vi "RemoteVI Hover Parent Menu.vi"(0 "hWnd":u64, 1 "now":u32, 5 "menus":T2(array[cluster]), 7 "k":i32=1, 9 "state":T1, 11 "error in":errorcluster) -> (4 "state out":T1, 15 "error out":errorcluster)   [LabVIEW 2020, in "RemoteVI.lvlib"]
doc: "The remote pointer rests over a PARENT menu (menus[k], k > 0) while k submenus are open below it - what happens locally when the pointer moves back from a submenu. When the pointer is on the parent's highlighted item (the one that opened the submenu) nothing changes and the submenu stays open. Otherwise, once the pointer has not moved for 300 ms (so a pointer crossing the parent on its way into the submenu does not close it), the k submenus are closed with VK_LEFT (RemoteVI Close Submenus.vi) and the parent's highlight is moved under the pointer (RemoteVI Hover Navigate.vi). Before that state passes through unchanged. Win32 only, no VI Server call."
uses:
  RemoteVI.lvlib
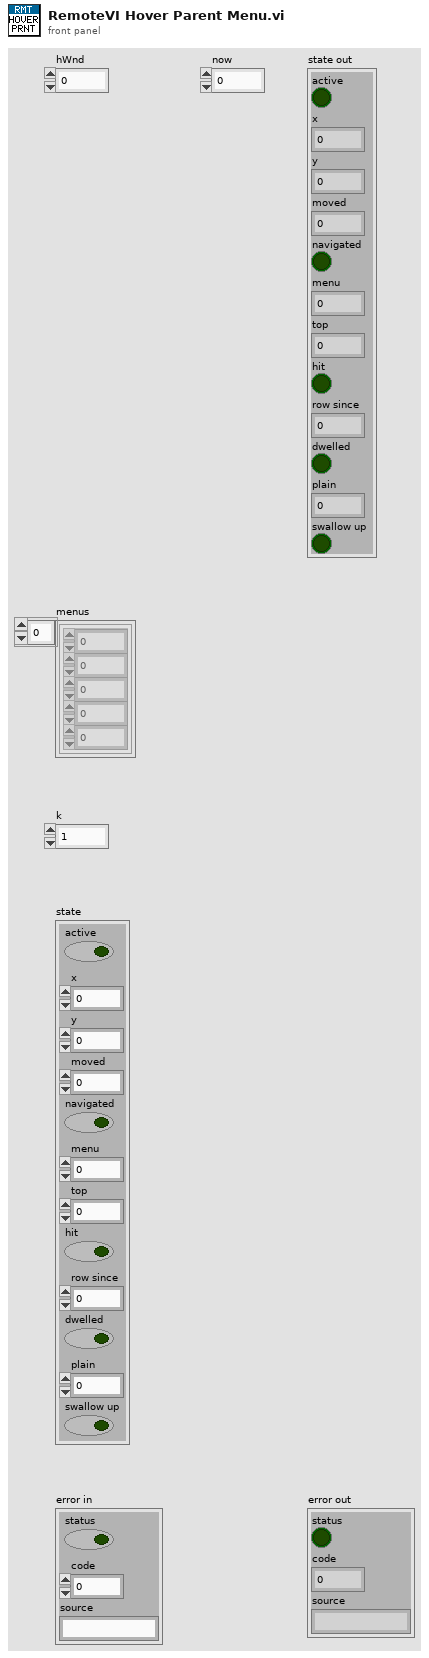
[diagram p1: front panel]
types:
  T1 = cluster{"active":bool, "x":i32, "y":i32, "moved":u32, "navigated":bool, "menu":u64, "top":i32, "hit":bool, "row since":u32, "dwelled":bool, "plain":u64, "swallow up":bool}
  T2 = cluster{"hwnd":u64, "x":i32, "y":i32, "w":i32, "h":i32}[]
  T3 = cluster{"hwnd":u64, "x":i32, "y":i32, "w":i32, "h":i32}
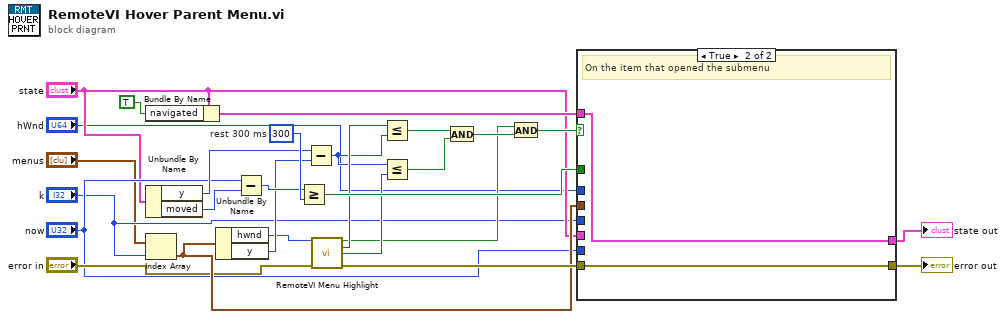
[diagram p0: block diagram]
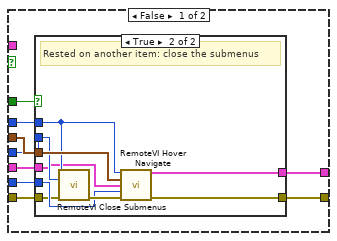
[diagram p2: hidden frame]
diagram:
  w22 = u32 300  # rest 300 ms
  n1 = Bundle By Name(cluster="state", "navigated"=TRUE) -> (w25:T1)
  n2 = Unbundle By Name("state") -> ("y"=w10:i32, "moved"=w11:u32)
  n3 = Index Array(array="menus", index="k") -> (element=w7:T3)
  n4 = Unbundle By Name(w7) -> ("hwnd"=w8:u64, "y"=w9:i32)
  n5 = Subtract(x="now", y=w11) -> (x-y=w21:u32)
  n6 = Greater Or Equal?(x=w21, y=w22) -> (x >= y?=w23:bool)
  n7 = Subtract(x=w10, y=w9) -> (x-y=w12:i32)
  n8 = call "RemoteVI Menu Highlight.vi"("hwnd"=w8, "error in"="error in") -> ("found?"=w13:bool, "top"=w14:i32, "bottom"=w15:i32, "error out"=w16:errorcluster)  [unwired: 7 in, 3 out]
  n9 = Less Or Equal?(x=w14, y=w12) -> (x <= y?=w17:bool)
  n10 = Less Or Equal?(x=w12, y=w15) -> (x <= y?=w18:bool)
  n11 = And(x=w17, y=w18) -> (x .and. y?=w19:bool)
  n12 = And(x=w13, y=w19) -> (x .and. y?=w20:bool)
  n13 = case shown="True" w20 {
    tunnel: "state" -> [w28 _]
    tunnel: "hWnd" -> [w31 _]
    tunnel: "k" -> [w32 _]
    tunnel: "now" -> [w34 _]
    tunnel: w25 -> [_ w48]
    tunnel: w7 -> [w33 _]
    tunnel: [w35 w48] -> w26
    tunnel: w16 -> [w29 w49]
    tunnel: w23 -> [w30 _]
    tunnel: [w36 w49] -> w27
    frame False {
      n14 = case shown="True" w30 {
        tunnel: w28 -> [w37 w39]
        tunnel: w31 -> [_ w41]
        tunnel: w32 -> [_ w42]
        tunnel: w34 -> [_ w44]
        tunnel: w33 -> [_ w43]
        tunnel: w29 -> [w38 w40]
        tunnel: [w37 w46] -> w35
        tunnel: [w38 w47] -> w36
        frame False {
        }
        frame True {
          # "Rested on another item: close the submenus"
          n15 = call "RemoteVI Close Submenus.vi"("hWnd"=w41, "count"=w42, "error in"=w40) -> ("error out"=w45:errorcluster)  [unwired: 12 in]
          n16 = call "RemoteVI Hover Navigate.vi"("hWnd"=w41, "menu"=w43, "state"=w39, "now"=w44, "error in"=w45) -> ("state out"=w46:T1, "error out"=w47:errorcluster)  [unwired: 9 in]
        }
      }
    }
    frame True {
      # "On the item that opened the submenu"
    }
  }
  "state out" <- w26
  "error out" <- w27
